vi "csb crc32.vi"(8 "error in (no error)":errorcluster, 10 "len":i32, 11 "data":u8[](array[numeric])) -> (0 "error out":errorcluster, 3 "function return":u32)   [LabVIEW 2021, in "CANsub_Codec.lvlib"]
doc: "uint32_t csb_crc32(const uint8_t *data, int32_t len);"
uses:
  CANsub_Codec.lvlib
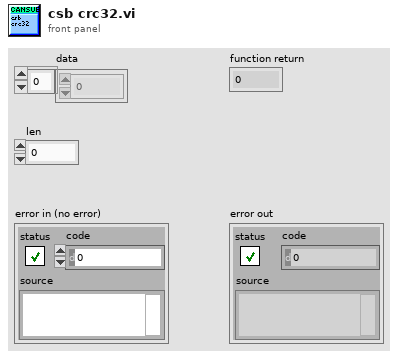
[diagram p1: front panel]
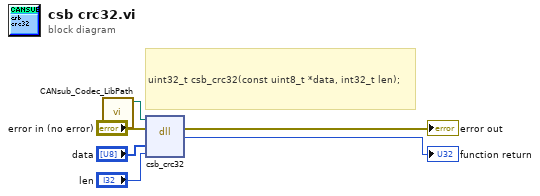
[diagram p0: block diagram]
diagram:
  # "uint32_t csb_crc32(const uint8_t *data, int32_t len);"
  n1 = call "CANsub_Codec_LibPath.vi"() -> ("Path"=w1:path)  [unwired: 11 in]
  n2 = dll-call lib="libcansub_codec.*" fn="csb_crc32"(path in=w1, error in="error in (no error)", "data"="data", "len"="len") -> (error out=→"error out":errorcluster, "return type"=→"function return":u32)  [unwired: 3 in, 1 out]
